vi "Write Double Direct.vi"(8 "error in (no error)":errorcluster, 10 "Data":dbl, 11 "CIFTag in":refnum<class "CIF_Iceoryx_Chn_Double.lvclass">) -> (0 "error out":errorcluster, 3 "CIFTag out":refnum<class "CIF_Iceoryx_Chn_Double.lvclass">)   [LabVIEW 2021, in "CIF_Iceoryx_Chn_Double.lvclass"]
uses:
  CIF_Iceoryx_Chn_Double.lvclass
  D:/dev/Packages/CIF_Channels_Core/src/Iceorxy_Channels/CIF_Iceoryx_BB/CIF_Iceoryx_BB.lvclass
  D:/dev/Packages/CIF_Channels_Core/src/CIFChannels/CIFChannels.lvclass
  CIF_Iceoryx_BB/CIF_Iceoryx_BB.lvclass/CIF_Iceoryx_BB.ctl
  CIFChannels/CIFChannels.lvclass/CIFChannels.ctl
  CIF_Iceoryx_Chn_Double.lvclass/CIF_Iceoryx_Chn_Double.ctl
  36393718-afdf-41a6-b430-da9823bc1f33.vi
  CIF_Iceoryx_BB/Accessors/Read Writer Reference.vi
  CIFChannels/Accessors/Read Tag Forced.vi
  <vilib>/CIF Foundation/CIF Iceoryx/SubVIs/Get Path.vi
  <vilib>/CIF Foundation/CIF Iceoryx/SubVIs/Convert Error.vi
  <vilib>/CIF Foundation/CIF Iceoryx/Refnum/BB Writer from Refnum.vi
  <vilib>/CIF Foundation/CIF Iceoryx/SubVIs/Convert Error Core.vi
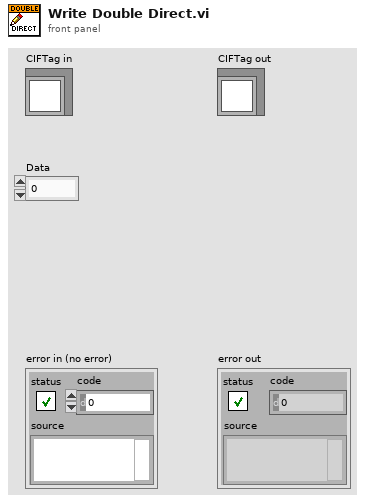
[diagram p1: front panel]
types:
  T1 = typedef "Iceoryx.lvlib/BB Writer Refnum.ctl" = cluster{"refnum":u64, "BB Writer":enum8{"bb_writer"}}
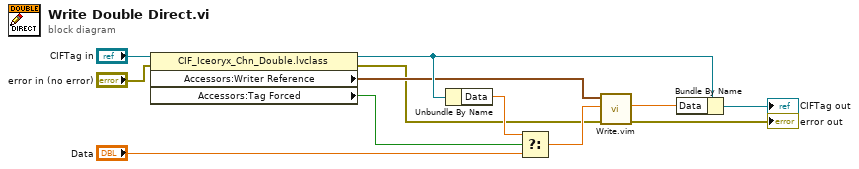
[diagram p0: block diagram]
diagram:
  n1 = property class="CIF_Iceoryx_Chn_Double.lvclass"(reference="CIFTag in", error in="error in (no error)") -> (reference out=w3:refnum<class "CIF_Iceoryx_Chn_Double.lvclass">, error out=w1:errorcluster, "Accessors:Writer Reference"=w2:T1, "Accessors:Tag Forced"=w4:bool)
  n2 = Unbundle By Name(w3) -> ("Data"=w7:dbl)
  n3 = Select(t=w7, s=w4, f="Data") -> (s? t:f=w6:dbl)
  n4 = call "Write.vim"("error in (no error)"=w1, "Data In"=w6, "Writer Reference"=w2) -> ("error out"=→"error out":errorcluster, "Data Out"=w5:dbl)  [unwired: 7 in]
  n5 = Bundle By Name(cluster=w3, "Data"=w5) -> (→"CIFTag out":refnum<class "CIF_Iceoryx_Chn_Double.lvclass">)
